vi "VM Spy - VM Datatype to List Symbol.vi"(11 "VarMan Datatype Code":u32) -> (3 "List/Tree Symbol":i32)   [LabVIEW 2021]
doc: "::: CalcExpress Toolkit :::\nCopyright (c) 2000-2026 Konstantin Shifershteyn. All rights reserved."
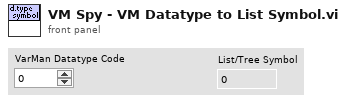
[diagram p1: front panel]
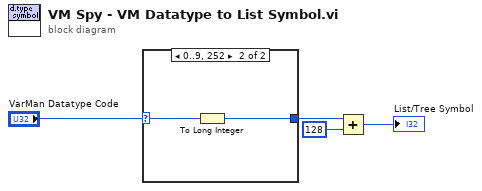
[diagram p0: block diagram]
diagram:
  n1 = case shown="0..9, 252" "VarMan Datatype Code" {
    selector: "VarMan Datatype Code" -> [_ w7]
    tunnel: [128 w6] -> w3
    frame Default {
    }
    frame 0..9, 252 {
      n2 = To Long Integer(number=w7) -> (32bit integer=w6:i32)
    }
  }
  n3 = Add(x=w3, y=128) -> (x+y=→"List/Tree Symbol":i32)
